vi "Connector Pane for Main Measurement.vi"(0 "VI in":refnum<vi>, 11 "error in":errorcluster) -> (4 "VI out":refnum<vi>, 15 "error out":errorcluster)   [LabVIEW 2021, in "Migrator.lvlib"]
uses:
  Migrator.lvlib
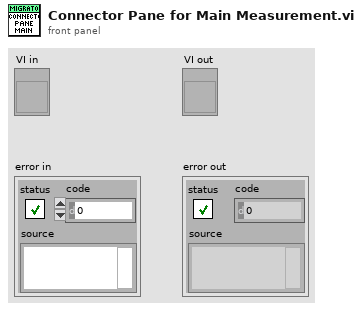
[diagram p1: front panel]
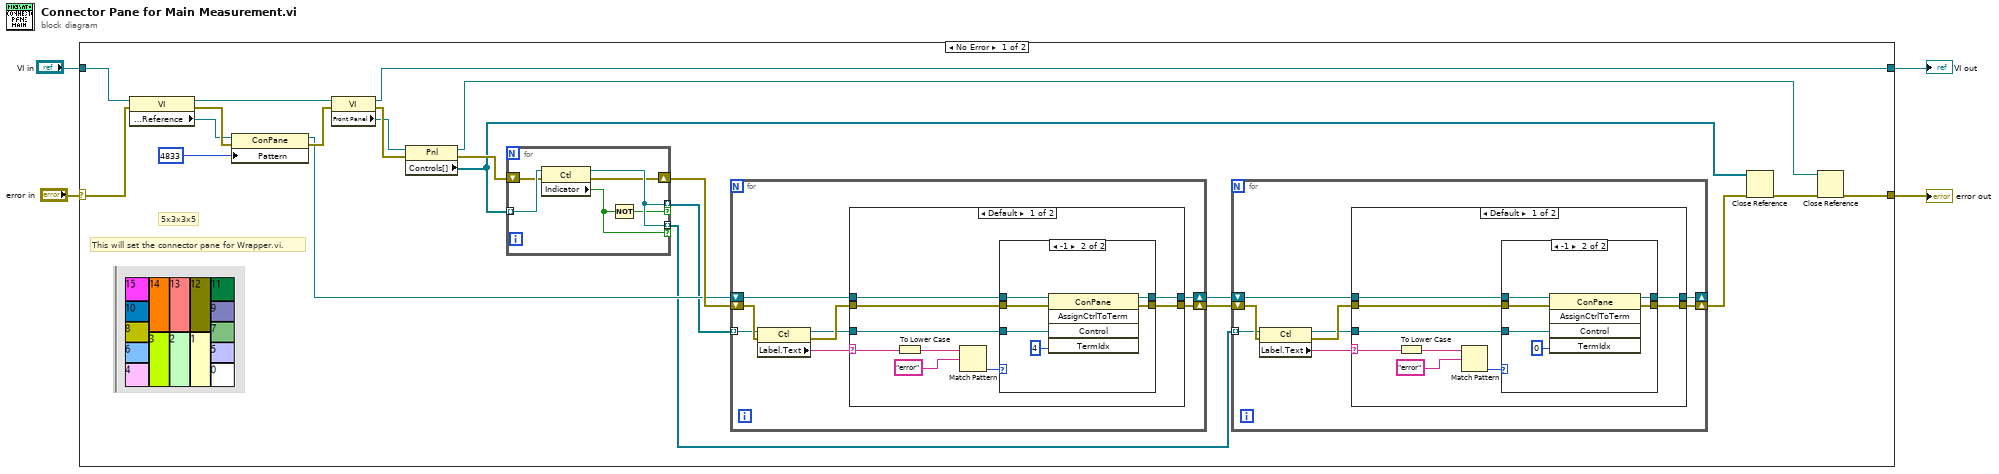
[diagram p0: block diagram]
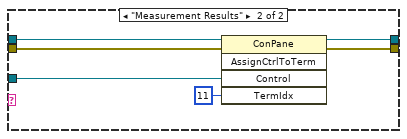
[diagram p3: hidden frame]
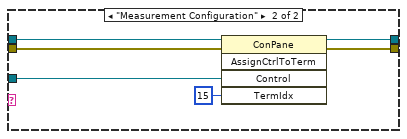
[diagram p5: hidden frame]
diagram:
  n1 = case shown="No Error" "error in" {
    selector: "error in" -> [w21 w96]
    tunnel: [w7 w96] -> w4
    tunnel: "VI in" -> [w20 w95]
    tunnel: [w5 w95] -> w1
    frame No Error {
      # "5x3x3x5"
      # "This will set the connector pane for Wrapper.vi."
      n2 = property class="VI"(reference=w20, error in=w21) -> (reference out=w22:refnum<vi>, error out=w25:errorcluster, "Connector Pane:Reference"=w23:refnum<vi>)
      n3 = property class="ConPane"(reference=w23, error in=w25, "Pattern"=u32 4833) -> (reference out=w15:refnum<vi>, error out=w24:errorcluster)
      n4 = property class="VI"(reference=w22, error in=w24) -> (reference out=w5:refnum<vi>, error out=w19:errorcluster, "Front Panel"=w17:refnum<vi>)
      n5 = property class="Pnl"(reference=w17, error in=w19) -> (reference out=w6:refnum<vi>, error out=w18:errorcluster, "Controls[]"=w8:refnum<vi>[])
      n6 = for {
        tunnel: w8 -> [w94] mode=indexing
        shift-right: [w89] -> w16
        shift-left: w18 -> [w93]
        tunnel: [w92] -> w11 mode=indexing if=w91
        tunnel: [w92] -> w14 mode=indexing if=w90
        n7 = property class="Ctl"(reference=w94, error in=w93) -> (reference out=w92:refnum<vi>, error out=w89:errorcluster, "Indicator"=w91:bool)
        n8 = Not(x=w91) -> (.not. x?=w90:bool)
      }
      n9 = for {
        tunnel: w14 -> [w62] mode=indexing
        shift-right: [w58] -> w12
        shift-left: w16 -> [w65]
        shift-right: [w59] -> w13
        shift-left: w15 -> [w64]
        n10 = property class="Ctl"(reference=w62, error in=w65) -> (reference out=w61:refnum<vi>, error out=w63:errorcluster, "Label.Text"=w60:string)
        n11 = case shown="Default" w60 {
          selector: w60 -> [w74 _]
          tunnel: w63 -> [w70 w88]
          tunnel: w64 -> [w69 w87]
          tunnel: w61 -> [w68 w86]
          tunnel: [w67 w83] -> w59
          tunnel: [w66 w84] -> w58
          frame Default {
            n12 = To Lower Case(string=w74) -> (all lower case string=w73:string)
            n13 = Match Pattern(string=w73, regular expression="error") -> (offset past match=w71:i32)  [unwired: 1 in, 3 out]
            n14 = case shown="-1" w71 {
              tunnel: w70 -> [w76 w81]
              tunnel: w69 -> [w75 w80]
              tunnel: w68 -> [_ w79]
              tunnel: [w75 w78] -> w67
              tunnel: [w76 w77] -> w66
              frame Default {
              }
              frame -1 {
                n15 = invoke class="ConPane" method="AssignCtrlToTerm"(reference=w80, error in=w81, "Control"=w79, "TermIdx"=u32 4 ("Terminal Index")) -> (reference out=w78:refnum<vi>, error out=w77:errorcluster)  [unwired: 1 in, 3 out]
              }
            }
          }
          frame "Measurement Configuration" {
            n16 = invoke class="ConPane" method="AssignCtrlToTerm"(reference=w87, error in=w88, "Control"=w86, "TermIdx"=u32 15 ("Terminal Index")) -> (reference out=w83:refnum<vi>, error out=w84:errorcluster)  [unwired: 1 in, 3 out]
          }
        }
      }
      n17 = for {
        tunnel: w11 -> [w31] mode=indexing
        shift-right: [w27] -> w10
        shift-left: w12 -> [w34]
        shift-right: [w28] -> _
        shift-left: w13 -> [w33]
        n18 = property class="Ctl"(reference=w31, error in=w34) -> (reference out=w30:refnum<vi>, error out=w32:errorcluster, "Label.Text"=w29:string)
        n19 = case shown="Default" w29 {
          selector: w29 -> [w43 _]
          tunnel: w32 -> [w39 w57]
          tunnel: w33 -> [w38 w56]
          tunnel: w30 -> [w37 w55]
          tunnel: [w36 w52] -> w28
          tunnel: [w35 w53] -> w27
          frame Default {
            n20 = To Lower Case(string=w43) -> (all lower case string=w42:string)
            n21 = Match Pattern(string=w42, regular expression="error") -> (offset past match=w40:i32)  [unwired: 1 in, 3 out]
            n22 = case shown="-1" w40 {
              tunnel: w39 -> [w45 w50]
              tunnel: w38 -> [w44 w49]
              tunnel: w37 -> [_ w48]
              tunnel: [w44 w47] -> w36
              tunnel: [w45 w46] -> w35
              frame Default {
              }
              frame -1 {
                n23 = invoke class="ConPane" method="AssignCtrlToTerm"(reference=w49, error in=w50, "Control"=w48, "TermIdx"=u32 0 ("Terminal Index")) -> (reference out=w47:refnum<vi>, error out=w46:errorcluster)  [unwired: 1 in, 3 out]
              }
            }
          }
          frame "Measurement Results" {
            n24 = invoke class="ConPane" method="AssignCtrlToTerm"(reference=w56, error in=w57, "Control"=w55, "TermIdx"=u32 11 ("Terminal Index")) -> (reference out=w52:refnum<vi>, error out=w53:errorcluster)  [unwired: 1 in, 3 out]
          }
        }
      }
      n25 = Close Reference(reference=w8, error in (no error)=w10) -> (error out=w9:errorcluster)
      n26 = Close Reference(reference=w6, error in (no error)=w9) -> (error out=w7:errorcluster)
    }
    frame Error {
    }
  }
  "error out" <- w4
  "VI out" <- w1
